vi "Initialize.vi"(8 "error in":errorcluster, 11 "Shared Resources in":refnum<class "Shared Resources.lvclass">) -> (0 "error out":errorcluster, 3 "Shared Resources out":refnum<class "Shared Resources.lvclass">)   [LabVIEW 2020, in "AIM ARINC 429 Engine.lvlib" / "Implementation.lvlib" / "Shared Resources.lvclass"]
uses:
  Shared Resources.lvclass
  Hardware API/AIM ARINC 429 Hardware API.lvlib
  <instrlib>/AIM GmbH/_ARINC-429/AIM429LV.lvlib
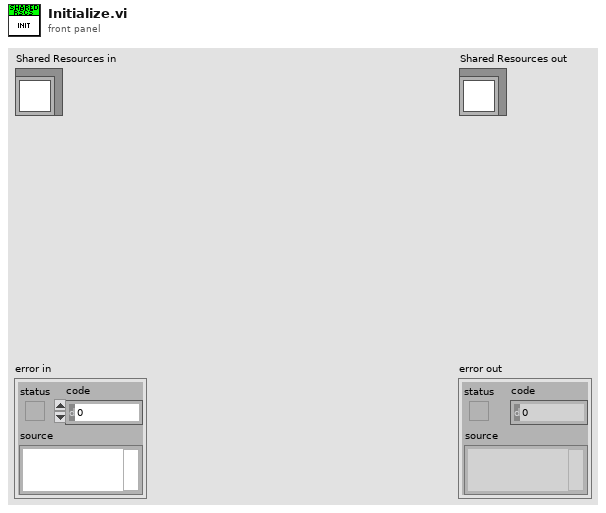
[diagram p1: front panel]
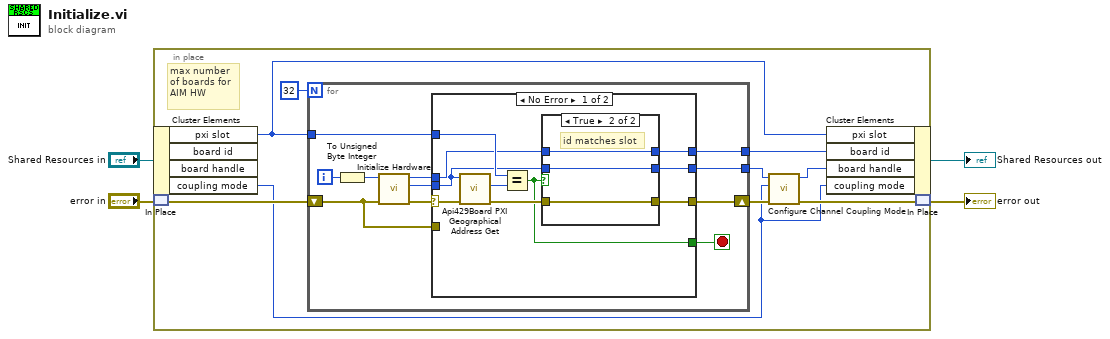
[diagram p0: block diagram]
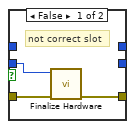
[diagram p2: hidden frame]
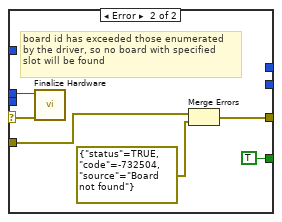
[diagram p3: hidden frame]
diagram:
  n1 = in-place {
    # "max number\nof boards for\nAIM HW"
    n2 = in-place-cluster #1("Shared Resources in") -> ("pxi slot"=w10:u8, "coupling mode"=w5:u32)  [unwired: 2 out]
    n3 = in-place-match #2("error in") -> (w13:errorcluster)
    n4 = for {
      N: 32 -> [_]
      shift-right: [w19] -> w9
      shift-left: w13 -> [w14]
      tunnel: w10 -> [w20]
      tunnel: [w17] -> w8
      tunnel: [w16] -> w11
      i -> [w24]
      stop <- w15 stop-if-true
      n5 = To Unsigned Byte Integer(number=w24) -> (unsigned 8bit integer=w23:u8)
      n6 = call "Initialize Hardware.vi"("error in"=w14, "board identifier in"=w23) -> ("error out"=w22:errorcluster, "module handle out"=w21:u8, "board identifier out"=w18:u8)  [unwired: 7 in]
      n7 = case shown="No Error" w22 {
        selector: w22 -> [w34 w46]
        tunnel: w21 -> [w31 _]
        tunnel: w20 -> [w32 _]
        tunnel: [w28 w41] -> w19
        tunnel: w18 -> [w27 w45]
        tunnel: [w30 _] -> w17
        tunnel: [w26 _] -> w16
        tunnel: [w25 TRUE] -> w15
        tunnel: w14 -> [_ w43]
        frame No Error {
          n8 = call <instrlib>:"Api429Board PXI Geographical Address Get.vi"("error in (no error)"=w34, "boardHandle"=w31) -> ("error out"=w29:errorcluster, "pxiSlotGeographicalAddress out"=w33:u32)  [unwired: 8 in]
          n9 = Equal?(x=w32, y=w33) -> (x = y?=w25:bool)
          n10 = case shown="True" w25 {
            tunnel: w31 -> [w36 w40]
            tunnel: [_ w40] -> w30
            tunnel: w29 -> [w37 w39]
            tunnel: [w35 w39] -> w28
            tunnel: w27 -> [_ w38]
            tunnel: [_ w38] -> w26
            frame False {
              # "not correct slot"
              n11 = call "Finalize Hardware.vi"("error in"=w37, "board identifier"=w36) -> ("error out"=w35:errorcluster)  [unwired: 9 in]
            }
            frame True {
              # "id matches slot"
            }
          }
        }
        frame Error {
          # "board id has exceeded those enumerated\nby the driver, so no board with specified\nslot will be found"
          n12 = call "Finalize Hardware.vi"("error in"=w46, "board identifier"=w45) -> ()  [unwired: 9 in, 1 out]
          n13 = Merge Errors(w43, errorcluster {"status"=TRUE, "code"=-732504, "source"="Board not found"} ("error in (no error)")) -> (w41:errorcluster)
        }
      }
    }
    n14 = call "Configure Channel Coupling Mode.vi"("error in"=w9, "coupling mode"=w5, "board handle"=w8) -> ("error out"=w6:errorcluster, "board handle out"=w7:u8)  [unwired: 7 in]
    n15 = in-place-cluster #1("pxi slot"=w10, "board id"=w11, "board handle"=w7, "coupling mode"=w5) -> (→"Shared Resources out":refnum<class "Shared Resources.lvclass">)
    n16 = in-place-match #2(w6) -> (→"error out":errorcluster)
  }
